vi "User.vi"   [LabVIEW 2019, in "xy_utilities.lvlib"]
doc: "Use for calling user code. Wire a User.lvclass to choose class instance.\n\nWire data to the data input to determine the polymorphic instance to use or manually select the instance."
uses:
  xy_utilities.lvlib
  User/User.lvclass
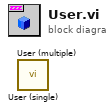
[diagram p0: block diagram]
diagram:
  n1 = call "User (single).vi"() -> ()  [unwired: 9 in, 3 out]
  n2 = call "User (multiple).vi"() -> ()  [unwired: 9 in, 3 out]
